vi "BNAL Intial txt and tdms tag_MS.vi"(6 "error in (no error)":errorcluster caption="error in", 8 "Level Composition":string[](array[string]), 9 "Date":string, 10 "Right Read MIN":i32, 11 "Folder Path":string) -> (1 "L_Tag cluster":T1, 3 "CSV_Path cluster":T2, 4 "error out":errorcluster, 5 "BS Table Tag":string[](array[string]))   [LabVIEW 2018]
panel:
  out "LAP_Tag":string[](array[string])
  out "size(s)":i32
  out "LTP Table Pass":path
  out "LTP Table Tag":string[](array[string])
  out "LCP Table Tag":string[](array[string])
  out "LSP Table Tag":string[](array[string])
  out "LCP Table Pass":path
  out "LSP Table Pass":path
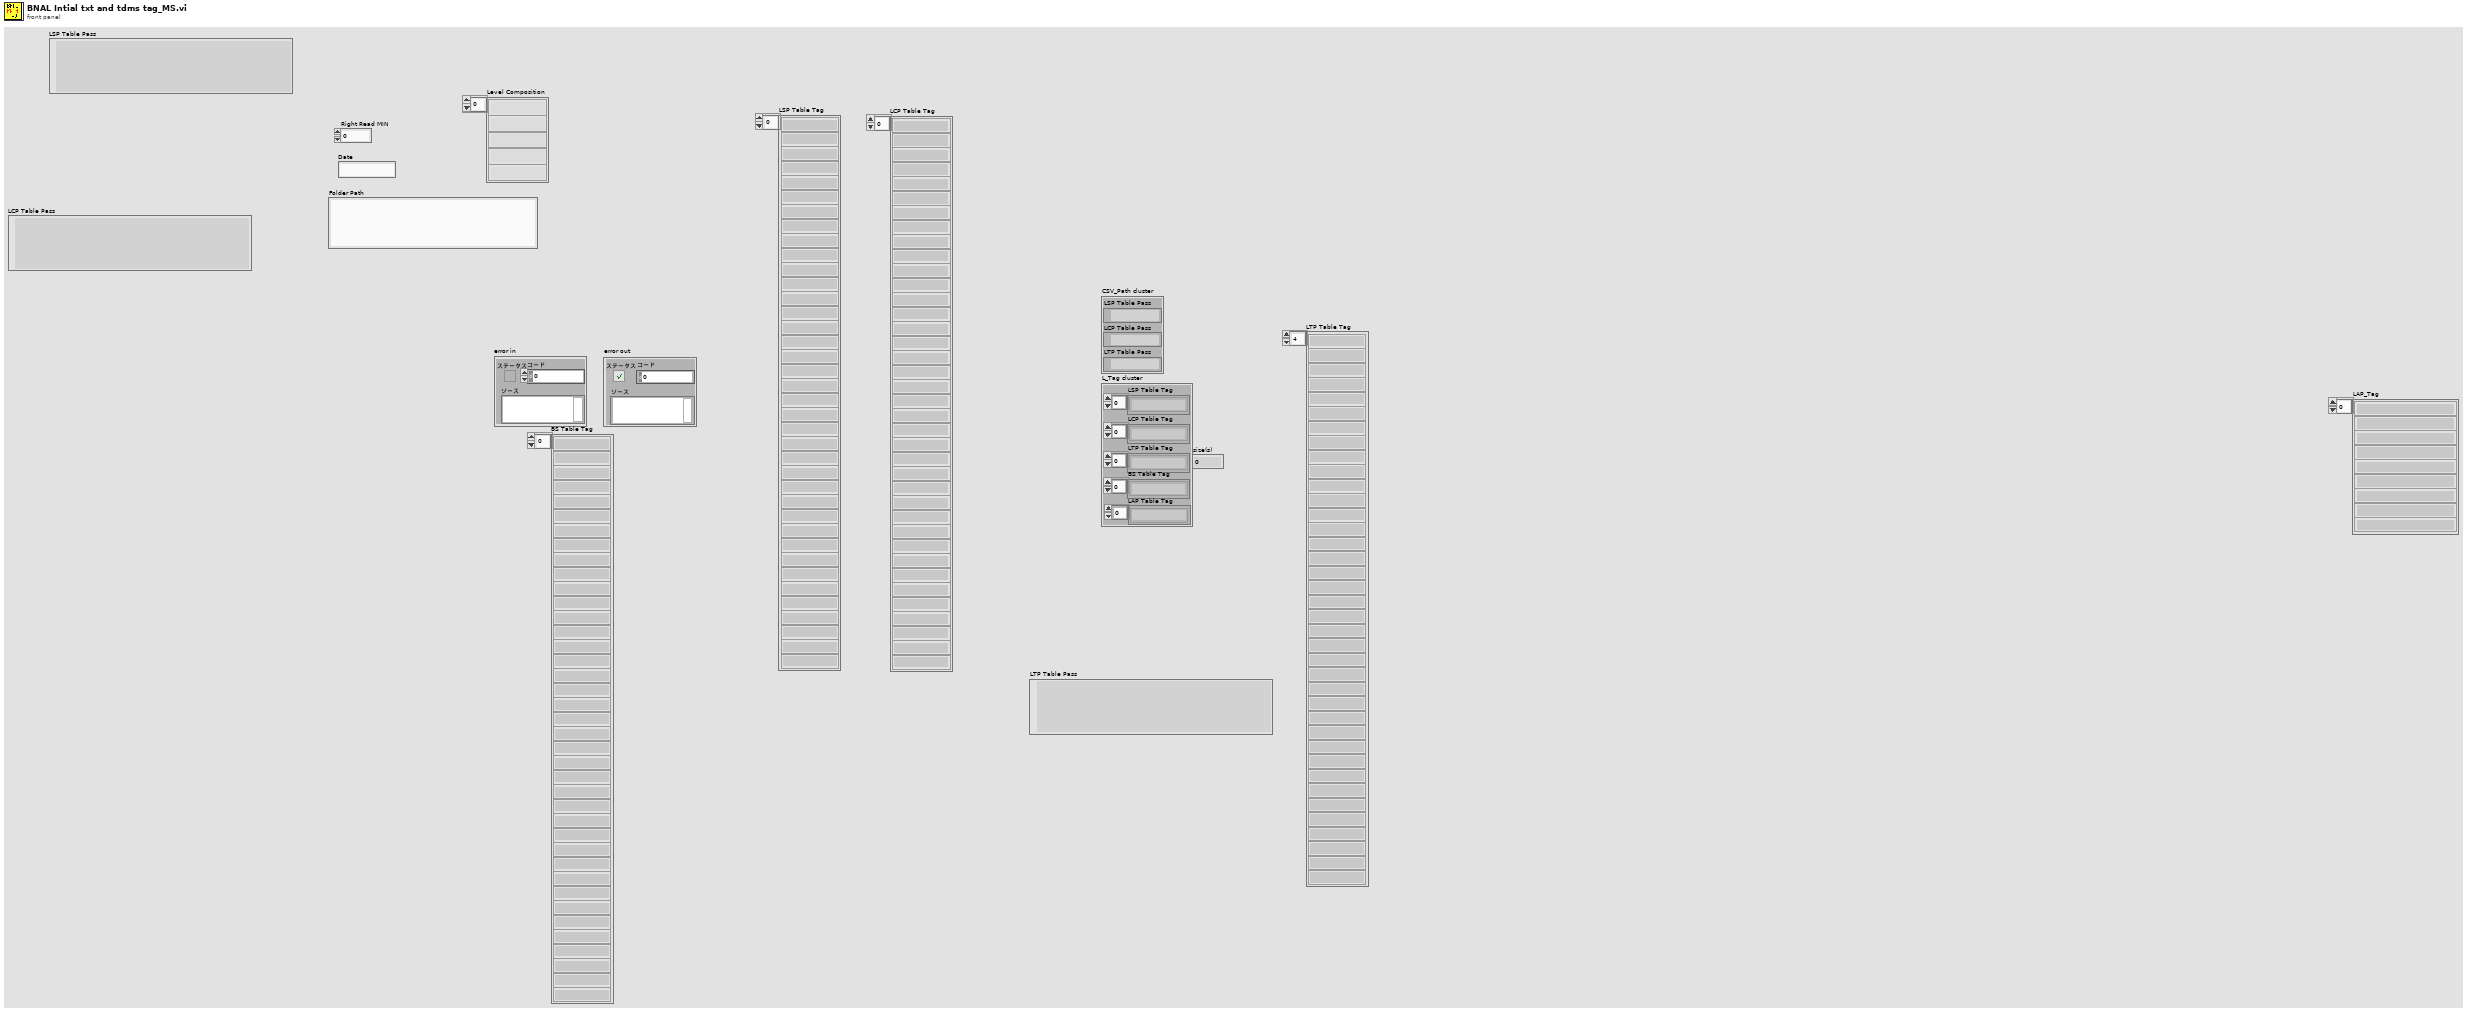
[diagram p1: front panel]
types:
  T1 = cluster{"LSP Table Tag":string[], "LCP Table Tag":string[], "LTP Table Tag":string[], "BS Table Tag":string[], "LAP Table Tag":string[]}
  T2 = cluster{"LSP Table Pass":path, "LCP Table Pass":path, "LTP Table Pass":path}
  T3 = cluster{"Value":string[], "Value":string[], "Value":string[], "Value":string[], "Value":string[]}
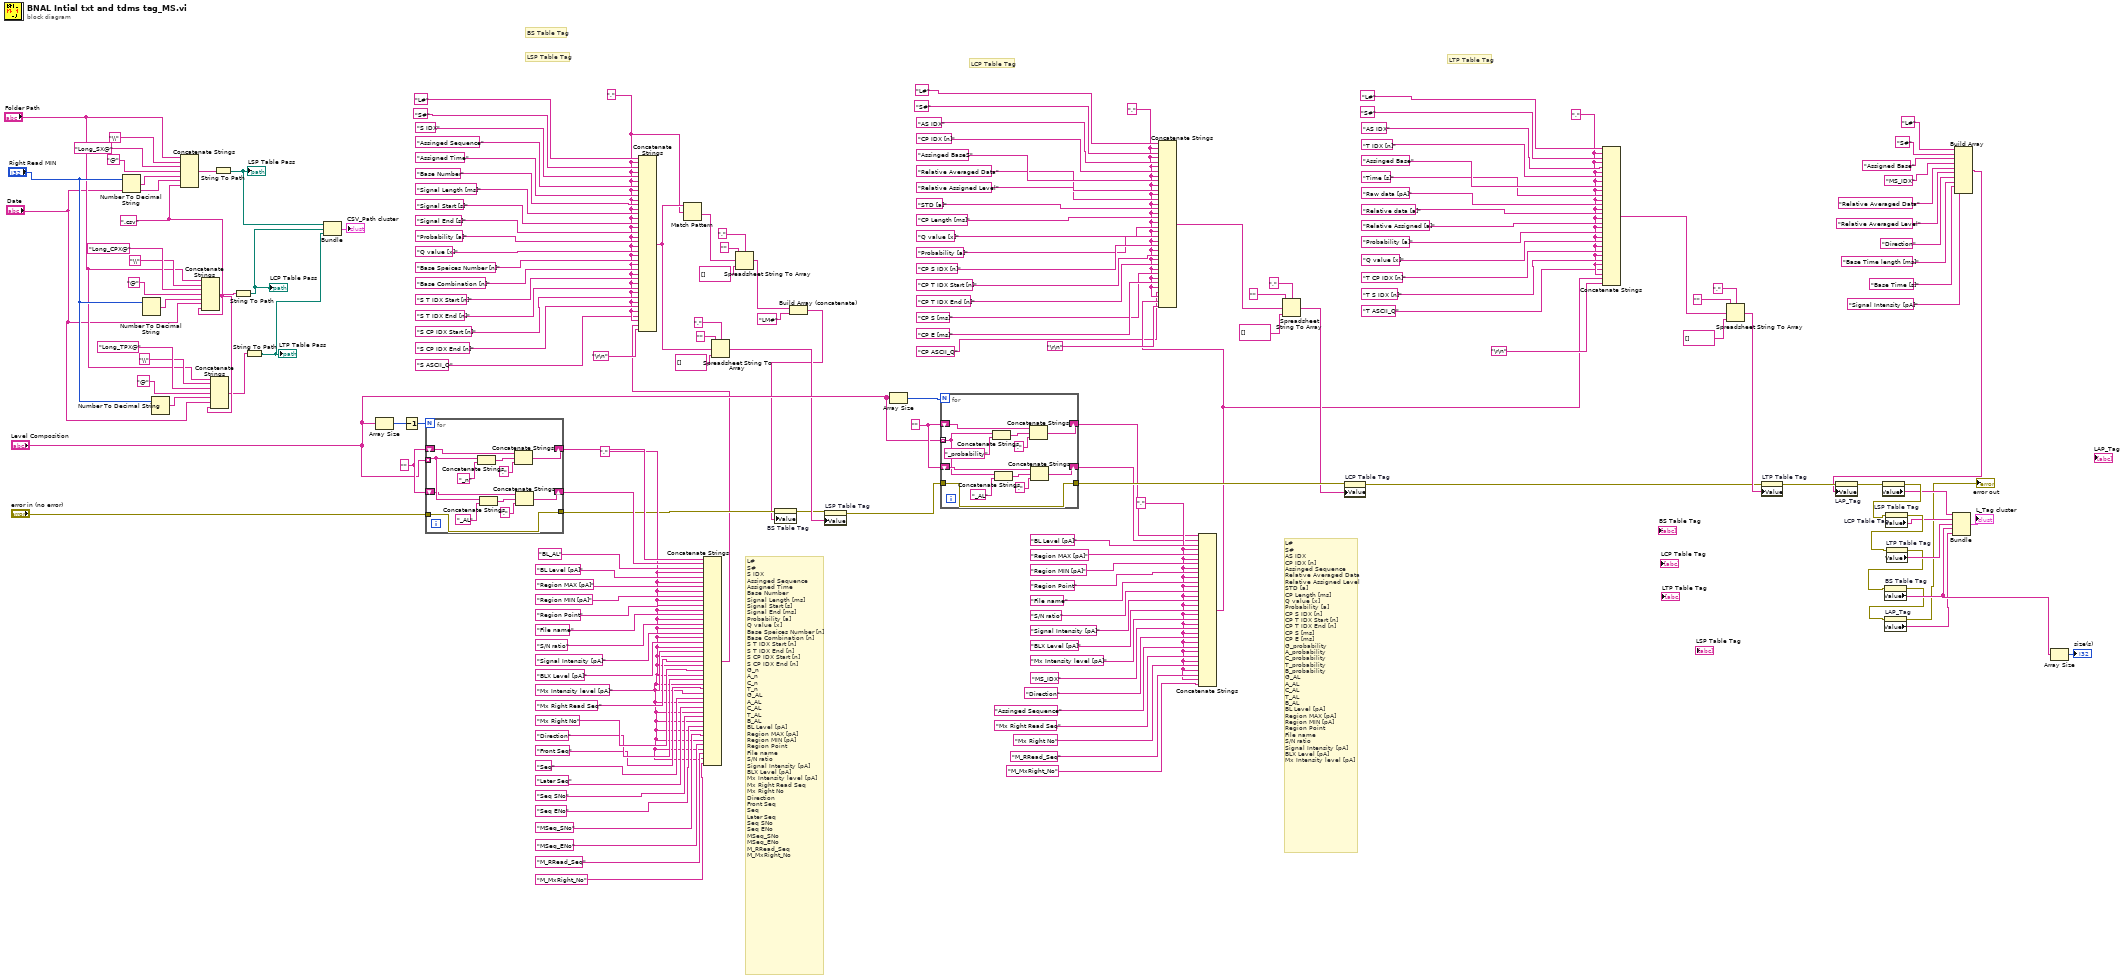
[diagram p0: block diagram]
diagram:
  w6 = "," ("デリミタ（タブ）")
  w82 = "," ("デリミタ（タブ）")
  w116 = ""
  w2 = "," ("デリミタ（タブ）")
  w90 = "," ("デリミタ（タブ）")
  w151 = ""
  w9 = "," ("デリミタ（タブ）")
  w59 = ".csv" ("文字列")
  # "LSP Table Tag"
  # "BS Table Tag"
  # "LCP Table Tag"
  # "LTP Table Tag"
  # "L#\nS#\nAS IDX\nCP IDX [n]\nAssinged Sequence\nRelative Averaged Data\nRelative Assigned Level\nSTD [a]\nCP Length [ms]\nQ value [x]\nProbability [a]\nCP S IDX [n]\nCP T IDX Start [n]\nCP T IDX End [n]\nCP S [ms]\nCP E [ms]\nG_probability\nA_probability\nC_probability\nT_probability\nB_probability\nG_AL\nA_AL\nC_AL\nT_AL\nB_AL\nBL Level [pA]\nRegion MAX [pA]\nRegion MIN [pA]\nRegion Point\nFile name\nS/N ratio\nSignal Intensity [pA]\nBLX Level [pA]\nMx Intensity level [pA]"
  # "L#\nS#\nS IDX\nAssinged Sequence\nAssigned Time\nBase Number\nSignal Length [ms]\nSignal Start [s]\nSignal End [ms]\nProbability [a]\nQ value [x]\nBase Speices Number [n]\nBase Combination [n]\nS T IDX Start [n]\nS T IDX End [n]\nS CP IDX Start [n]\nS CP IDX End [n]\nG_n\nA_n\nC_n\nT_n\nG_AL\nA_AL\nC_AL\nT_AL\nB_AL\nBL Level [pA]\nRegion MAX [pA]\nRegion MIN [pA]\nRegion Point\nFile name\nS/N ratio\nSignal Intensity [pA]\nBLX Level [pA]\nMx Intensity level [pA]\nMx Right Read Seq\nMx Right No\nDirection\nFront Seq\nSeq\nLater Seq\nSeq SNo\nSeq ENo\nMSeq_SNo\nMSeq_ENo\nM_RRead_Seq\nM_MxRight_No"
  n1 = Number To Decimal String(number="Right Read MIN") -> (decimal integer string=w180:string)  [unwired: 1 in]
  n2 = Number To Decimal String(number="Right Read MIN") -> (decimal integer string=w175:string)  [unwired: 1 in]
  n3 = Number To Decimal String(number="Right Read MIN") -> (decimal integer string=w64:string)  [unwired: 1 in]
  n4 = Concatenate Strings("Folder Path", "\\" ("文字列"), "Long_SX@" ("LG name"), "@" ("文字列"), w180, "Date", w59) -> (w182:string)
  n5 = Concatenate Strings("Folder Path", "\\" ("文字列"), "Long_CPX@" ("LG name"), "@" ("文字列"), w175, "Date", w59) -> (w177:string)
  n6 = Concatenate Strings("Folder Path", "\\" ("文字列"), "Long_TPX@" ("LG name"), "@" ("文字列"), w64, "Date", w59) -> (w58:string)
  n7 = String To Path(string=w182) -> (path=w56:path)
  "LSP Table Pass" <- w56
  n8 = String To Path(string=w177) -> (path=w55:path)
  "LCP Table Pass" <- w55
  n9 = String To Path(string=w58) -> (path=w54:path)
  "LTP Table Pass" <- w54
  n10 = Bundle(w56, w55, w54) -> (→"CSV_Path cluster":cluster{path, path, path})  [unwired: 1 in]
  n11 = Array Size(array="Level Composition") -> (size(s)=w157:i32)
  n12 = Decrement(x=w157) -> (x-1=w158:i32)
  n13 = for {
    N: w158 -> [_]
    tunnel: "Level Composition" -> [w187] mode=indexing
    shift-right: [w193] -> w103
    shift-left: w151 -> [w192]
    shift-right: [w186] -> w104
    shift-left: w151 -> [w185]
    tunnel: "error in (no error)" -> [w184]
    tunnel: [w184] -> w53
    n14 = Concatenate Strings(w187, "_n" ("文字列")) -> (w195:string)
    n15 = Concatenate Strings(w187, "_AL" ("文字列")) -> (w190:string)
    n16 = Concatenate Strings(w192, w195, "," ("デリミタ（タブ）")) -> (w193:string)
    n17 = Concatenate Strings(w185, w190, "," ("デリミタ（タブ）")) -> (w186:string)
  }
  n18 = Concatenate Strings(w103, w104, "BL_AL" ("書き込みバッファ"), w90, "BL Level [pA]" ("書き込みバッファ"), w90, "Region MAX [pA]" ("書き込みバッファ"), w90, "Region MIN [pA]" ("書き込みバッファ"), w90, "Region Point" ("書き込みバッファ"), w90, "File name" ("書き込みバッファ"), w90, "S/N ratio" ("書き込みバッファ"), w90, "Signal Intensity [pA]" ("書き込みバッファ"), w90, "BLX Level [pA]" ("書き込みバッファ"), w90, "Mx Intensity level [pA]" ("書き込みバッファ"), w90, "Mx Right Read Seq" ("文字列"), w90, "Mx Right No" ("文字列"), w90, "Direction" ("文字列"), w90, "Front Seq" ("文字列"), w90, "Seq" ("文字列"), w90, "Later Seq" ("文字列"), w90, "Seq SNo" ("文字列"), w90, "Seq ENo" ("文字列"), w90, "MSeq_SNo" ("文字列"), w90, "MSeq_ENo" ("文字列"), w90, "M_RRead_Seq" ("文字列"), w90, "M_MxRight_No" ("文字列")) -> (w10:string)
  n19 = Concatenate Strings("L#" ("文字列"), w9, "S#" ("書き込みバッファ"), w9, "S IDX" ("文字列"), w9, "Assinged Sequence" ("書き込みバッファ"), w9, "Assigned Time" ("書き込みバッファ"), w9, "Base Number" ("書き込みバッファ"), w9, "Signal Length [ms]" ("書き込みバッファ"), w9, "Signal Start [s]" ("書き込みバッファ"), w9, "Signal End [s]" ("書き込みバッファ"), w9, "Probability [a]" ("書き込みバッファ"), w9, "Q value [x]" ("書き込みバッファ"), w9, "Base Speices Number [n]" ("書き込みバッファ"), w9, "Base Combination [n]" ("書き込みバッファ"), w9, "S T IDX Start [n]" ("書き込みバッファ"), w9, "S T IDX End [n]" ("書き込みバッファ"), w9, "S CP IDX Start [n]" ("書き込みバッファ"), w9, "S CP IDX End [n]" ("書き込みバッファ"), w9, "S ASCII_Q" ("書き込みバッファ"), w9, w10, "\r\n") -> (w99:string)
  n20 = Match Pattern(string=w99, regular expression=w9) -> (after substring=w95:string)  [unwired: 1 in, 3 out]
  n21 = Spreadsheet String To Array(delimiter (Tab)="," ("デリミタ（タブ）"), format string="" ("形式文字列"), spreadsheet string=w99, array type (2D Dbl)=string[] [] ("行ヘッダ文字列[]")) -> (array=w41:string[])
  n22 = Spreadsheet String To Array(delimiter (Tab)="," ("デリミタ（タブ）"), format string="" ("形式文字列"), spreadsheet string=w95, array type (2D Dbl)=string[] [] ("行ヘッダ文字列[]")) -> (array=w32:string[])
  n23 = Build Array (concatenate)(w32, "LM#" ("形式文字列")) -> (w31:string[])
  n24 = property on="BS Table Tag" class="Arr (strict)"(error in=w53, "Value"=w31) -> (error out=w40:errorcluster)  [unwired: 1 in, 1 out]
  n25 = property on="LSP Table Tag" class="Arr (strict)"(error in=w40, "Value"=w41) -> (error out=w39:errorcluster)  [unwired: 1 in, 1 out]
  n26 = Array Size(array="Level Composition") -> (size(s)=w44:i32)
  n27 = for {
    N: w44 -> [_]
    shift-right: [w205] -> w42
    shift-left: w116 -> [w204]
    shift-right: [w199] -> w43
    shift-left: w116 -> [w198]
    tunnel: "Level Composition" -> [w197] mode=indexing
    tunnel: w39 -> [w196]
    tunnel: [w196] -> w52
    n28 = Concatenate Strings(w197, "_probability" ("文字列")) -> (w207:string)
    n29 = Concatenate Strings(w197, "_AL" ("文字列")) -> (w202:string)
    n30 = Concatenate Strings(w204, w207, "," ("デリミタ（タブ）")) -> (w205:string)
    n31 = Concatenate Strings(w198, w202, "," ("デリミタ（タブ）")) -> (w199:string)
  }
  n32 = Concatenate Strings(w42, w43, "BL Level [pA]" ("書き込みバッファ"), w82, "Region MAX [pA]" ("書き込みバッファ"), w82, "Region MIN [pA]" ("書き込みバッファ"), w82, "Region Point" ("書き込みバッファ"), w82, "File name" ("書き込みバッファ"), w82, "S/N ratio" ("書き込みバッファ"), w82, "Signal Intensity [pA]" ("書き込みバッファ"), w82, "BLX Level [pA]" ("書き込みバッファ"), w82, "Mx Intensity level [pA]" ("書き込みバッファ"), w82, "MS_IDX" ("y"), w82, "Direction" ("y"), w82, "Assinged Sequence" ("y"), w82, "Mx Right Read Seq" ("y"), w82, "Mx Right No" ("y"), w82, "M_RRead_Seq" ("y"), w82, "M_MxRight_No" ("y")) -> (w3:string)
  n33 = Concatenate Strings("L#" ("文字列"), w2, "S#" ("書き込みバッファ"), w2, "AS IDX" ("書き込みバッファ"), w2, "CP IDX [n]" ("文字列"), w2, "Assinged BaseS" ("書き込みバッファ"), w2, "Relative Averaged Data" ("書き込みバッファ"), w2, "Relative Assigned Level" ("書き込みバッファ"), w2, "STD [a]" ("書き込みバッファ"), w2, "CP Length [ms]" ("書き込みバッファ"), w2, "Q value [x]" ("書き込みバッファ"), w2, "Probability [a]" ("書き込みバッファ"), w2, "CP S IDX [n]" ("書き込みバッファ"), w2, "CP T IDX Start [n]" ("書き込みバッファ"), w2, "CP T IDX End [n]" ("書き込みバッファ"), w2, "CP S [ms]" ("書き込みバッファ"), w2, "CP E [ms]" ("書き込みバッファ"), w2, "CP ASCII_Q" ("書き込みバッファ"), w2, w3, "\r\n") -> (w117:string)
  n34 = Spreadsheet String To Array(delimiter (Tab)="," ("デリミタ（タブ）"), format string="" ("形式文字列"), spreadsheet string=w117, array type (2D Dbl)=string[] [] ("行ヘッダ文字列[]")) -> (array=w51:string[])
  n35 = property on="LCP Table Tag" class="Arr (strict)"(error in=w52, "Value"=w51) -> (error out=w49:errorcluster)  [unwired: 1 in, 1 out]
  n36 = Concatenate Strings("L#" ("文字列"), w6, "S#" ("書き込みバッファ"), w6, "AS IDX" ("書き込みバッファ"), w6, "T IDX [n]" ("文字列"), w6, "Assinged Base" ("書き込みバッファ"), w6, "Time [s]" ("書き込みバッファ"), w6, "Raw data [pA]" ("書き込みバッファ"), w6, "Relative data [a]" ("書き込みバッファ"), w6, "Relative Assigned [a]" ("書き込みバッファ"), w6, "Probability [a]" ("書き込みバッファ"), w6, "Q value [x]" ("書き込みバッファ"), w6, "T CP IDX [n]" ("書き込みバッファ"), w6, "T S IDX [n]" ("書き込みバッファ"), w6, "T ASCII_Q" ("書き込みバッファ"), w6, w3, "\r\n") -> (w70:string)
  n37 = Spreadsheet String To Array(delimiter (Tab)="," ("デリミタ（タブ）"), format string="" ("形式文字列"), spreadsheet string=w70, array type (2D Dbl)=string[] [] ("行ヘッダ文字列[]")) -> (array=w50:string[])
  n38 = property on="LTP Table Tag" class="Arr (strict)"(error in=w49, "Value"=w50) -> (error out=w16:errorcluster)  [unwired: 1 in, 1 out]
  n39 = Build Array("L#" ("y"), "S#" ("y"), "Assigned Base" ("y"), "MS_IDX" ("y"), "Relative Averaged Data" ("y"), "Relative Averaged Level" ("y"), "Direction" ("y"), "Base Time length [ms]" ("y"), "Base Time [s]" ("y"), "Signal Intensity [pA]" ("y")) -> (w14:string[])
  n40 = property on="LAP_Tag" class="Arr (strict)"(error in=w16, "Value"=w14) -> (error out=w15:errorcluster)  [unwired: 1 in, 1 out]
  n41 = property on="LSP Table Tag" class="Arr (strict)"(error in=w15) -> (error out=w38:errorcluster, "Value"=w37:string[])  [unwired: 1 in, 1 out]
  n42 = property on="LCP Table Tag" class="Arr (strict)"(error in=w38) -> (error out=w48:errorcluster, "Value"=w47:string[])  [unwired: 1 in, 1 out]
  n43 = property on="LTP Table Tag" class="Arr (strict)"(error in=w48) -> (error out=w36:errorcluster, "Value"=w46:string[])  [unwired: 1 in, 1 out]
  n44 = property on="BS Table Tag" class="Arr (strict)"(error in=w36) -> (error out=w13:errorcluster, "Value"=w29:string[])  [unwired: 1 in, 1 out]
  n45 = property on="LAP_Tag" class="Arr (strict)"(error in=w13) -> (error out=→"error out":errorcluster, "Value"=w17:string[])  [unwired: 1 in, 1 out]
  n46 = Bundle("Value"=w37, "Value"=w47, "Value"=w46, "Value"=w29, "Value"=w17) -> (→"L_Tag cluster":T3)  [unwired: 1 in]
  n47 = Array Size(array=w29) -> (size(s)=→"size(s)":i32)
